vi "get network adapter settings.vi"(8 "error in":errorcluster, 11 "system session in":refnum<k21>) -> (0 "error out":errorcluster, 1 "secondary network adapters":T1[](array[typedef]) {"IP address request mode" items=["Static"=1, "DHCP/Link Local"=2, "Link-Local Only"=4, "DHCP Only"=8]; "adapter type" items=["Ethernet"=1, "WLAN"=2]; "adapter mode" items=["Disabled"=1, "TCP/IP Ethernet"=2, "Deterministic"=4, "EtherCAT"=8, "TCP/IP WLAN Connect"=32, "TCP/IP WLAN Create"=64]}, 2 "primary network adapter":T1 {"IP address request mode" items=["Static"=1, "DHCP/Link Local"=2, "Link-Local Only"=4, "DHCP Only"=8]; "adapter type" items=["Ethernet"=1, "WLAN"=2]; "adapter mode" items=["Disabled"=1, "TCP/IP Ethernet"=2, "Deterministic"=4, "EtherCAT"=8, "TCP/IP WLAN Connect"=32, "TCP/IP WLAN Create"=64]}, 3 "system session out":refnum<k21>)   [LabVIEW 2014, in "SMI.lvlib" / "Controller.lvclass"]
uses:
  Controller.lvclass
  network adapter settings.ctl
  <vilib>/nisyscfg/Close (Hardware).vi
  <vilib>/nisyscfg/Find Hardware.vi
  <vilib>/nisyscfg/nisyscfg.lvlib
  <resource>/objmgr/niflexriosae.rc
  SMI.lvlib
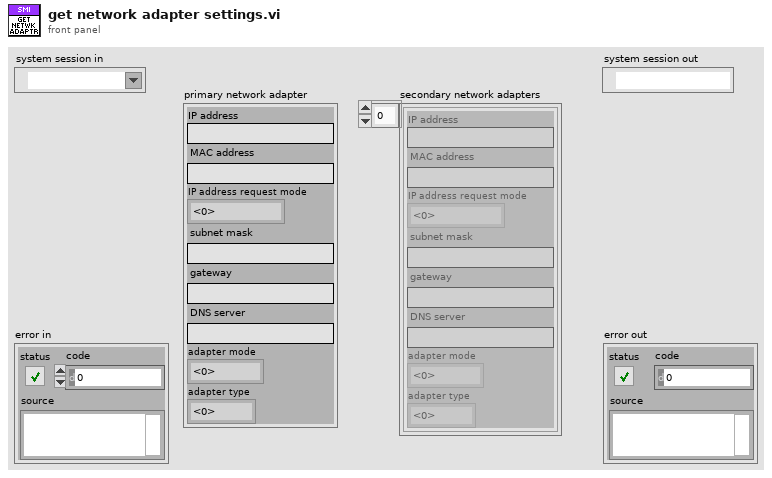
[diagram p1: front panel]
types:
  T1 = typedef "SMI.lvlib/Controller.lvclass/network adapter settings.ctl" = cluster{"IP address":string, "MAC address":string, "IP address request mode":u32, "subnet mask":string, "gateway":string, "DNS server":string, "adapter mode":u32, "adapter type":u32}
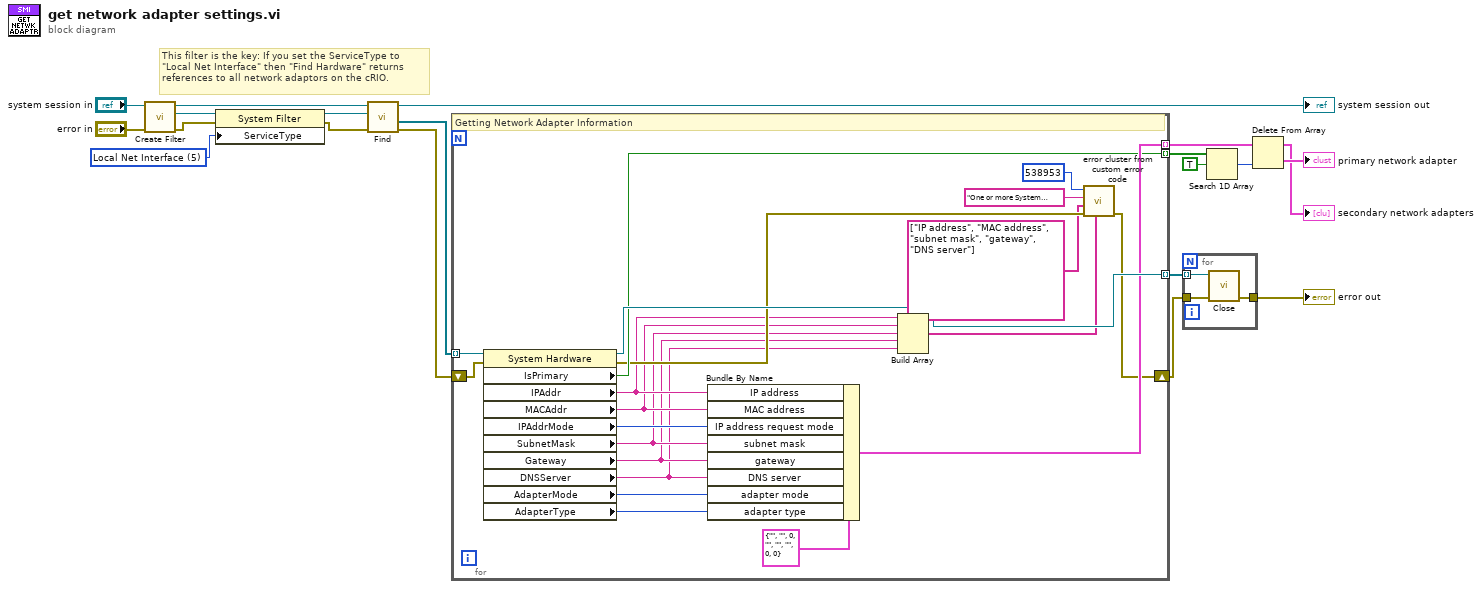
[diagram p0: block diagram]
diagram:
  w13 = u32 5 items=["NI Network Resource", "NI Real-Time", "NI System Configuration", "NI Web Interface", "Local System", "Local Net Interface", "Local Time Keeper", "Local Time Reference", "LXI Instrument"] ("Service Type")
  # "This filter is the key: If you set the ServiceType to\n\"Local Net Interface\" then \"Find Hardware\" returns\nreferences to all network adaptors on the cRIO."
  n1 = call <vilib>:"Create Filter.vi"("error in (no error)"="error in", "Session in"="system session in") -> ("error out"=w16:errorcluster, "Filter out"=w12:refnum<k20>, "Session out"=w11:refnum<k21>)  [unwired: 7 in]
  n2 = property class="System Filter"(reference=w12, error in=w16, "ServiceType"=w13) -> (reference out=w14:refnum<k20>, error out=w15:errorcluster)
  n3 = call-poly <vilib>:"Find.vi"("error in (no error)"=w15, "Filter in"=w14, "Session in"=w11) -> ("error out"=w17:errorcluster, "Resources out"=w7:refnum<k20>[], "Session out"=→"system session out":refnum<k21>)  [unwired: 5 in, 1 out]
  n4 = for {
    tunnel: w7 -> [w39] mode=indexing
    shift-right: [w31] -> w20
    shift-left: w17 -> [w40]
    tunnel: [w38] -> w10 mode=indexing
    tunnel: [w33] -> w6 mode=indexing
    tunnel: [w32] -> w5 mode=indexing
    # "Getting Network Adapter Information"
    n5 = property class="System Hardware"(reference=w39, error in=w40) -> (reference out=w38:refnum<k20>, error out=w30:errorcluster, "IsPrimary"=w32:bool, "IPAddr"=w29:string, "MACAddr"=w28:string, "IPAddrMode"=w36:u32, "SubnetMask"=w27:string, "Gateway"=w26:string, "DNSServer"=w25:string, "AdapterMode"=w35:u32, "AdapterType"=w34:u32)
    n6 = Bundle By Name(cluster=T1 {"IP address"="", "MAC address"="", "IP address request mode"=0, "subnet mask"="", "gateway"="", "DNS server"="", "adapter mode"=0, "adapter type"=0} ("Network Adapter Settings"), "IP address"=w29, "MAC address"=w28, "IP address request mode"=w36, "subnet mask"=w27, "gateway"=w26, "DNS server"=w25, "adapter mode"=w35, "adapter type"=w34) -> (w33:T1)
    n7 = Build Array(w29, w28, w27, w26, w25) -> (w22:string[])
    n8 = call "error cluster from custom error code.vi"("string values"=w22, "error in"=w30, "keys"=string[] ["IP address", "MAC address", "subnet mask", "gateway", "DNS server"], "error message"="One or more System Hardware properties are not available for one or more of the target network adapters.", "custom error code (0)"=538953 ("error code (0)")) -> ("error out"=w31:errorcluster)  [unwired: 6 in]
  }
  n9 = for {
    tunnel: [w43] -> w19
    tunnel: w20 -> [w42]
    tunnel: w10 -> [w41] mode=indexing
    n10 = call-poly <vilib>:"Close.vi"("error in (no error)"=w42, "Resource in"=w41) -> ("error out"=w43:errorcluster)  [unwired: 9 in]
  }
  "error out" <- w19
  n11 = Search 1D Array(1D array=w5, element=TRUE) -> (index of element=w3:i32)  [unwired: 1 in]
  n12 = Delete From Array(array=w6, index=w3) -> (deleted portion=→"primary network adapter":T1, array with subset deleted=→"secondary network adapters":T1[])  [unwired: 1 in]
